vi "Watchdog Add Restart RTE Action.vi"(4 "error in (no error)":errorcluster, 7 "watchdogID in":u64 format="%.0x") -> (0 "error out":errorcluster, 3 "watchdogID out":u64 format="%.0x")   [LabVIEW 2025]
doc: "<p>Configures the <a href=\"nihelplauncher://docs/csh?context=lvrt_lvrtconcepts_rt_watchdog\">watchdog object</a> to restart only the LabVIEW Run-Time Engine when the watchdog timer expires, without resetting the FPGA application or losing network connection. Use this VI in the configuration stage of the application, prior to the Watchdog Enable VI.</p>"
uses:
  niwd4c.dll
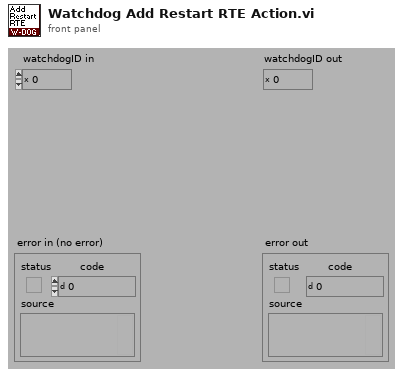
[diagram p1: front panel]
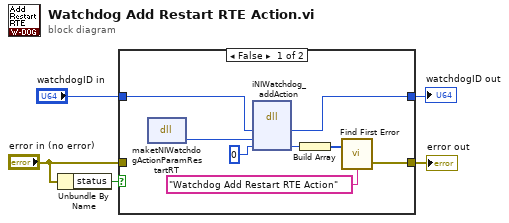
[diagram p0: block diagram]
diagram:
  n1 = Unbundle By Name("error in (no error)") -> ("status"=w5:bool)
  n2 = case shown="False" w5 {
    tunnel: [w8 w14] -> w2
    tunnel: [w12 w15] -> w1
    tunnel: "error in (no error)" -> [_ w15]
    tunnel: "watchdogID in" -> [w6 w14]
    frame False {
      n3 = dll-call lib="niwd4c.*" fn="maketNIWatchdogActionParamRestartRT" label="Action Restart RTE"() -> ("return type"=w10:u64)  [unwired: 3 in, 2 out]
      n4 = dll-call lib="niwd4c.*" fn="iNIWatchdog_addAction" label="Add Action"("wd"=w6, "parameter"=w10, "status"=0) -> ("wd"=w8:u64, "status"=w9:i32)  [unwired: 5 in, 2 out]
      n5 = Build Array(w9) -> (w13:i32[])
      n6 = call <vilib>:"Find First Error.vi"("source messages"="Watchdog Add Restart RTE Action", "error codes"=w13) -> ("error out"=w12:errorcluster)  [unwired: 2 in, 1 out]
    }
    frame True {
    }
  }
  "error out" <- w1
  "watchdogID out" <- w2
